vi "HostMem CopyToArray_1D-U16.vi"(8 "error in (no error)":errorcluster, 11 "HostMem in":refnum<class "HostMem.lvclass">) -> (0 "error out":errorcluster, 2 "Array":u16[](array[numeric]), 3 "HostMem out":refnum<class "HostMem.lvclass">)   [LabVIEW 2020, in "OpenLvVision_OpenCv.lvlib" / "Cuda.lvlib" / "HostMem.lvclass"]
doc: "Copies the hostmat data into an array."
uses:
  HostMem.lvclass
  C:/Users/lukas/Downloads/OpenLvVision_OpenCv/SourceCode/LabView/OpenLvVision_OpenCv/_LvHelpers/EdvrObject/EdvrObject.lvclass
  _LvHelpers/EdvrObject/EdvrObject.lvclass/EdvrObject.ctl
  _LvHelpers/MatHandling/RegisterMat/RegisterMat_Array1D-U16.vi
  OpenLvVision_OpenCv.lvlib
  _LvHelpers/EdvrObject/EdvrObject.lvclass
  <vilib>/Utility/error.llb/Error Cluster From Error Code.vi
  <vilib>/ErrorRing/Error Ring.xnode
  Dlls/OlvOpenCvWrapper.dll
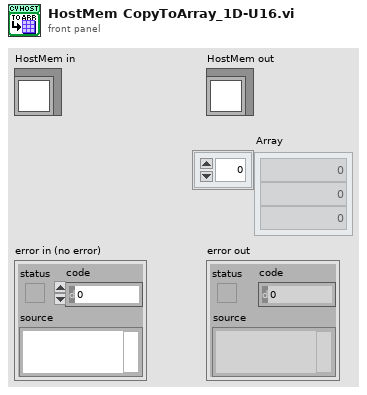
[diagram p1: front panel]
types:
  T1 = typedef "OpenLvVision_OpenCv.lvlib/HostMatInfo.ctl" = cluster{"Rows":i32, "Cols":i32, "cvType":T2, "Channels":i32, "depth":i32}
  T2 = typedef "OpenLvVision_OpenCv.lvlib/cvType.ctl" = enum32{"CV_8UC1", "CV_8SC1", "CV_16UC1", "CV_16SC1", "CV_32SC1", "CV_32FC1", "CV_64FC1", "CV_16FC1", "CV_8UC2", "CV_8SC2", "CV_16UC2", "CV_16SC2", "CV_32SC2", "CV_32FC2", "CV_64FC2", "CV_16FC2", "CV_8UC3", "CV_8SC3", "CV_16UC3", "CV_16SC3", "CV_32SC3", "CV_32FC3", "CV_64FC3", "CV_16FC3", "CV_8UC4", "CV_8SC4", "CV_16UC4", "CV_16SC4", "CV_32SC4", "CV_32FC4", "CV_64FC4", "CV_16FC4"}
  T3 = typedef "OpenLvVision_OpenCv.lvlib/MatInfo.ctl" = cluster{"Datatype":T4, "Height":i32, "Width":i32, "Channels":i32, "LineWidth":i32, "Null":u8}
  T4 = typedef "OpenLvVision_OpenCv.lvlib/LvDatatype.ctl" = enum32{"Undefined", "U8", "I8", "U16", "I16", "U32_Color", "I32", "U64_Color", "I64", "SGL", "DBL", "Complex SGL", "Complex DBL", "Array 1D U8", "Array 1D I8", "Array 1D U16", "Array 1D I16", "Array 1D U32_Color", "Array 1D I32", "Array 1D U64_Color", "Array 1D I64", "Array 1D SGL", "Array 1D DBL", "Array 1D Complex SGL", "Array 1D Complex DBL", "Array 2D U8", "Array 2D I8", "Array 2D U16", "Array 2D I16", "Array 2D U32", "Array 2D U32_Color", "Array 2D I32", "Array 2D U64", "Array 2D U64_Color", "Array 2D I64", "Array 2D SGL", "Array 2D DBL", "Array 2D Complex SGL", "Array 2D Complex DBL", "Image Mono U8", "Image Mono U16", "Image Mono I16", "Image Mono SGL", "Image Color U32", "Image Color U64", "ImageComplex Sgl", "Array1d_2dPointI32", "Array1d_2dPointSGL", "Array1d_2dPointDBL", "Array1d_3dPointI32", "Array1d_3dPointSGL", "Array1d_3dPointDBL", "Array1d_4dPointI32", "Array1d_4dPointSGL", "Array1d_4dPointDBL", "ArrayNchwU8", "ArrayNchwI8", "ArrayNchwU16", "ArrayNchwI16", "ArrayNchwU32_Color", "ArrayNchwI32", "ArrayNchwU64_Color", "ArrayNchwSgl", "ArrayNchwDbl", "ArrayNchwComplexSgl", "ArrayNchwComplexDbl"}
  T5 = typedef "OpenLvVision_OpenCv.lvlib/EdvrObject.lvclass/Edvr.ctl" = refnum<data-value>
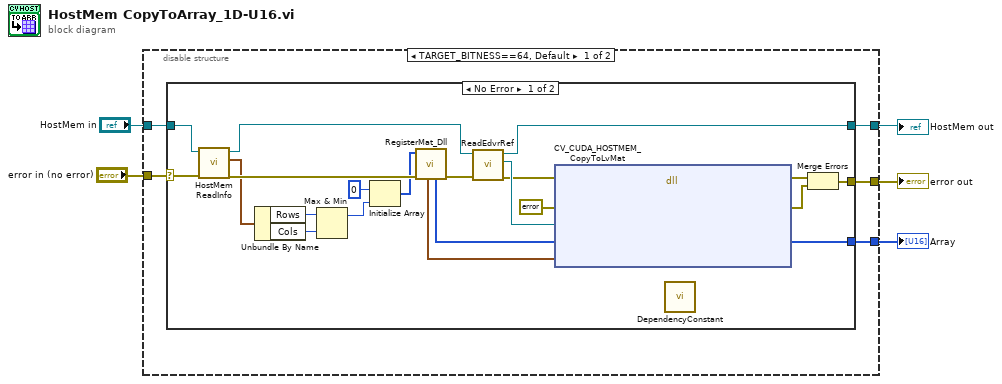
[diagram p0: block diagram]
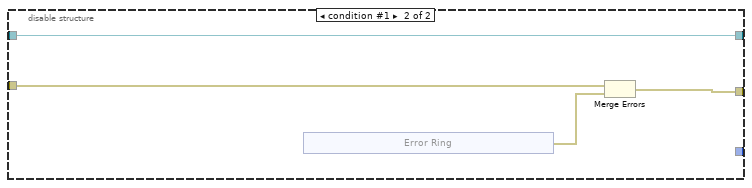
[diagram p3: hidden frame]
diagram:
  n1 = disable-structure shown="TARGET_BITNESS==64, Default" {
    disable-tunnel: "error in (no error)" -> [w10 w36]
    disable-tunnel: [w9 w37] -> w2
    disable-tunnel: "HostMem in" -> [w8 w34]
    disable-tunnel: [w7 w34] -> w3
    disable-tunnel: [w6 _] -> w1
    frame condition #0 (active) {
      n2 = case shown="No Error" w10 {
        selector: w10 -> [w23 w33]
        tunnel: [w22 w33] -> w9
        tunnel: w8 -> [w26 w32]
        tunnel: [w27 w32] -> w7
        tunnel: [w11 _] -> w6
        frame No Error {
          n3 = call "HostMem ReadInfo.vi"("error in (no error)"=w23, "HostMem in"=w26) -> ("error out"=w18:errorcluster, "HostMatInfo"=w15:T1, "HostMem out"=w25:refnum<class "HostMem.lvclass">)  [unwired: 7 in]
          n4 = Unbundle By Name(w15) -> ("Rows"=w13:i32, "Cols"=w14:i32)
          n5 = Max & Min(x=w13, y=w14) -> (max(x,y)=w12:i32)  [unwired: 1 out]
          n6 = Initialize Array(u16 0 ("element"), w12) -> (w16:u16[])
          n7 = call-poly "RegisterMat_Dll.vi"("error in"=w18, "Array in"=w16) -> ("error out"=w21:errorcluster, "AdressOrData"=w20:u16[], "Mat"=w19:T3)  [unwired: 6 in, 1 out]
          n8 = call "ReadEdvrRef.vi"("error in (no error)"=w21, "EdvrObject in"=w25) -> ("error out"=w24:errorcluster, "Edvr"=w28:T5, "EdvrObject out"=w27:refnum<class "HostMem.lvclass">)  [unwired: 7 in]
          n9 = dll-call lib="C:/Users/lukas/Downloads/OpenLvVision_OpenCv/SourceCode/LabView/OpenLvVision_OpenCv/Dlls/OlvOpenCvWrapper.dll" fn="CV_CUDA_HOSTMEM_CopyToLvMat"(error in=w24, "Error"=errorcluster {"status"=FALSE, "code"=0, "source"=""} ("error out"), "edvrRef"=w28, "addressDst"=w20, "matInfoDst"=w19) -> (error out=w31:errorcluster, "Error"=w30:errorcluster, "addressDst"=w11:u16[])  [unwired: 5 in, 1 out]
          n10 = call "DependencyConstant.vi"() -> ()  [unwired: 12 in]
          n11 = Merge Errors(w31, w30) -> (w22:errorcluster)
        }
        frame Error {
        }
      }
    }
    frame condition #1 {
      n12 = xnode "Error Ring"() -> ("error out"=w35:errorcluster)
      n13 = Merge Errors(w36, w35) -> (w37:errorcluster)
    }
  }
  "error out" <- w2
  "HostMem out" <- w3
  "Array" <- w1
